vi "Main_State_Machine.vi"   [LabVIEW 2026]
uses:
  Typedefs/System_State.ctl
  Typedefs/BeltCtrl.ctl
  Globals.vi
types:
  T1 = enum16{"open", "replace", "create", "open or create", "replace or create", "replace or create with confirmation"}
  T2 = typedef "System_State.ctl" = u16
  T3 = typedef "BeltCtrl.ctl" = enum16{"Off", "Forward", "Back", "Coast", "Brake", ""}
  T4 = typedef "ServoCommand.ctl" = enum16{"colour 1", "Colour2", "Colour3", "Reject"}
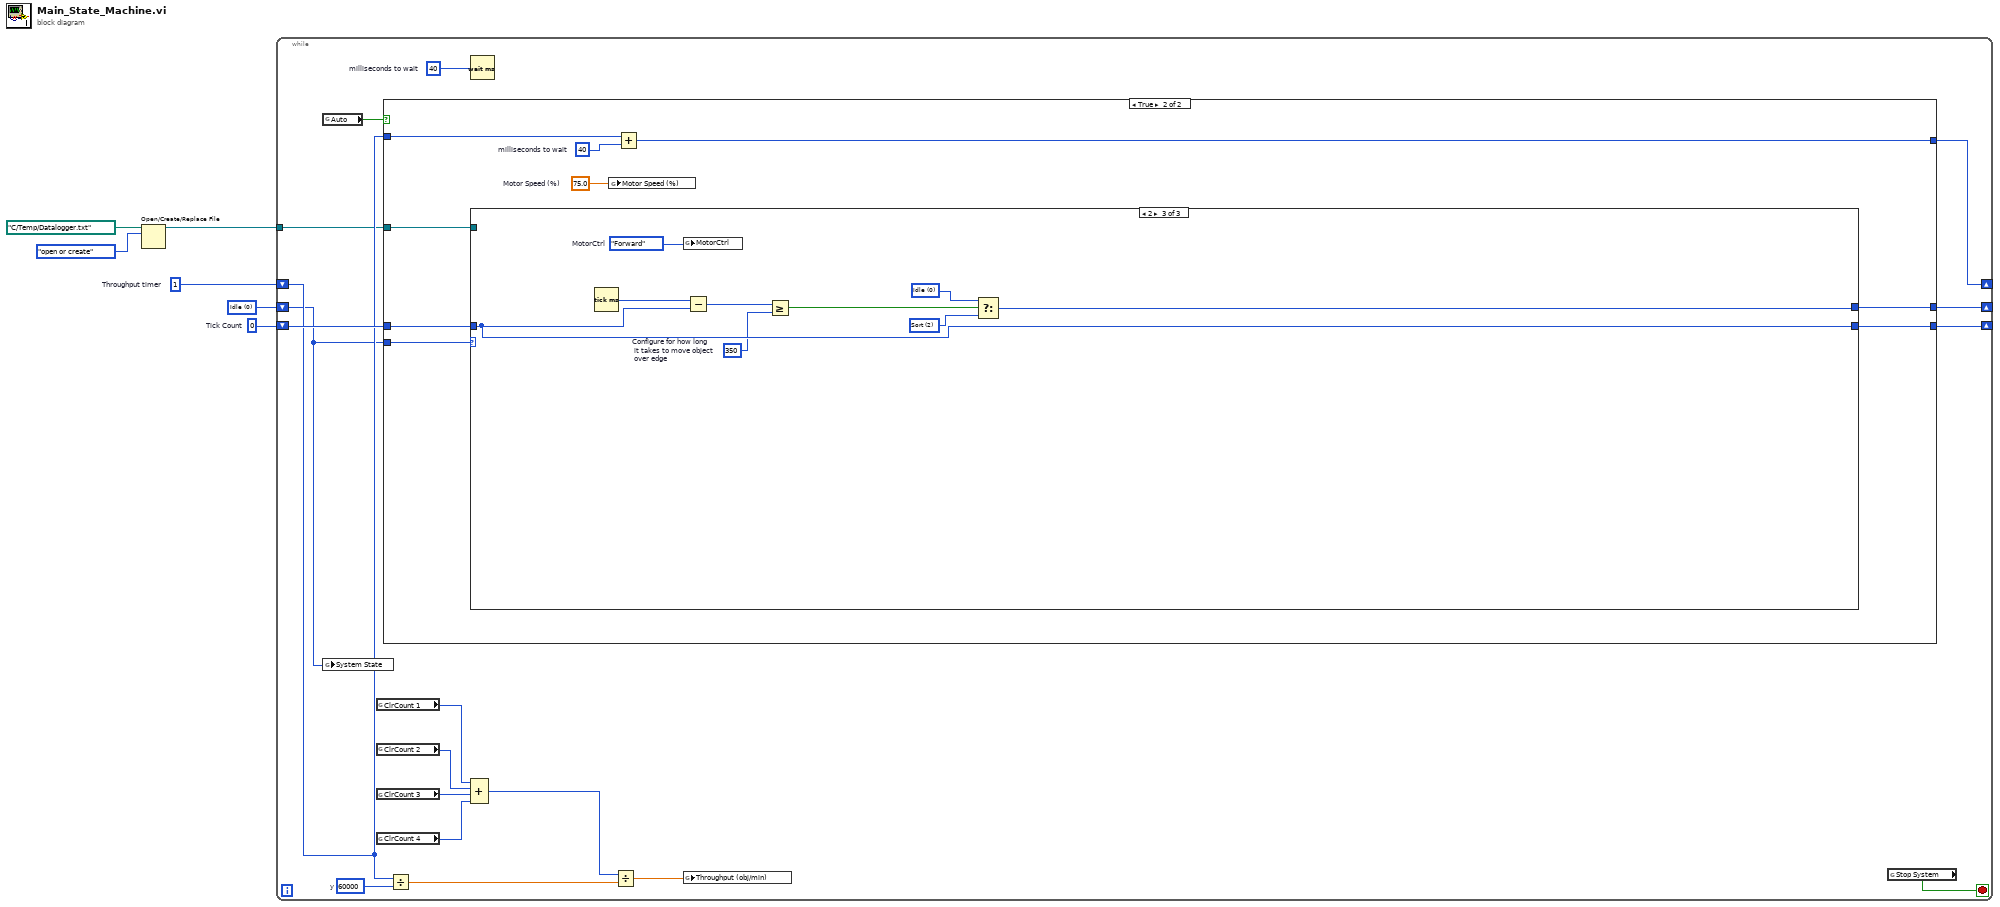
[diagram p0: block diagram]
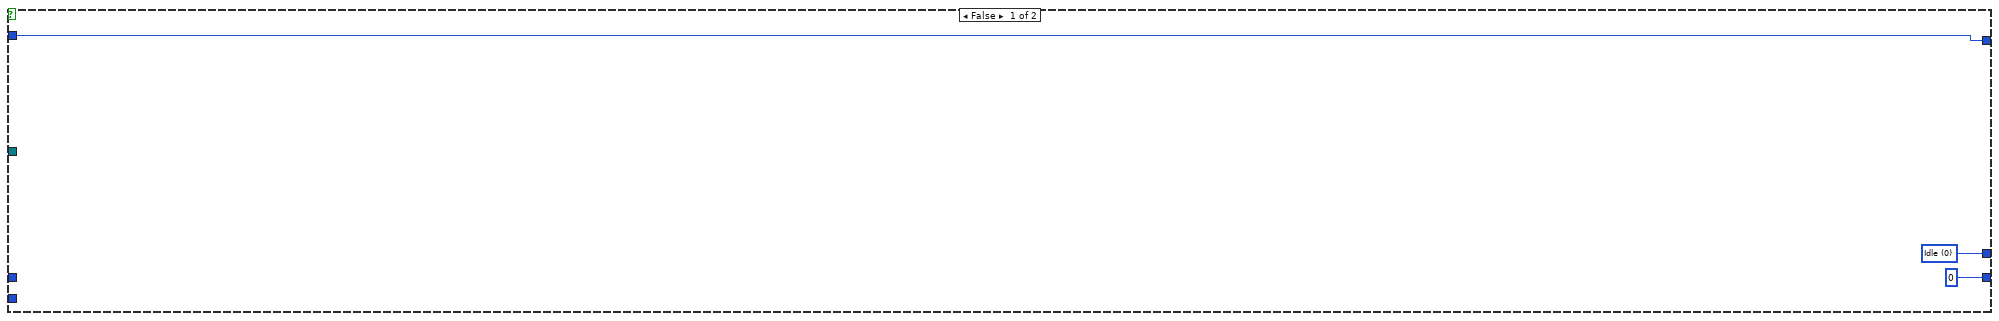
[diagram p2: hidden frame]
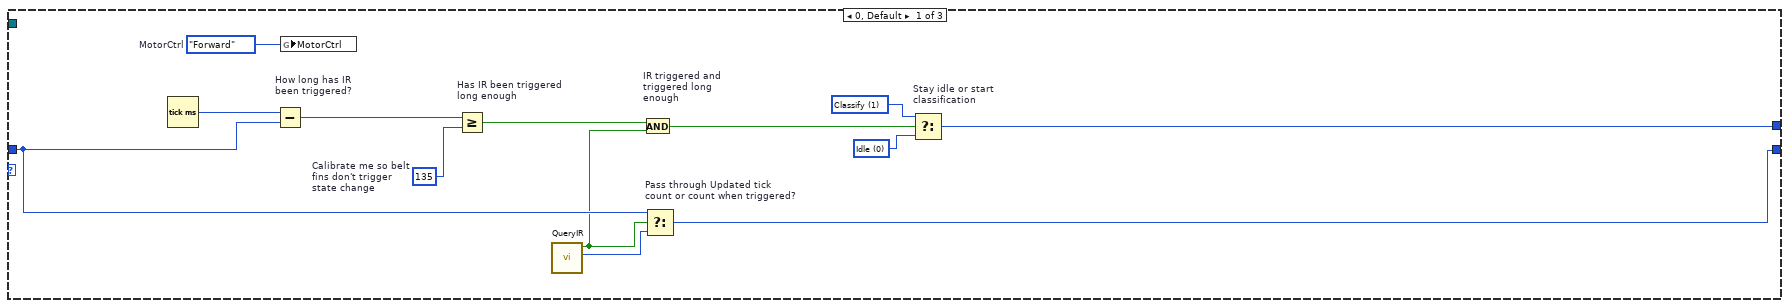
[diagram p3: hidden frame]
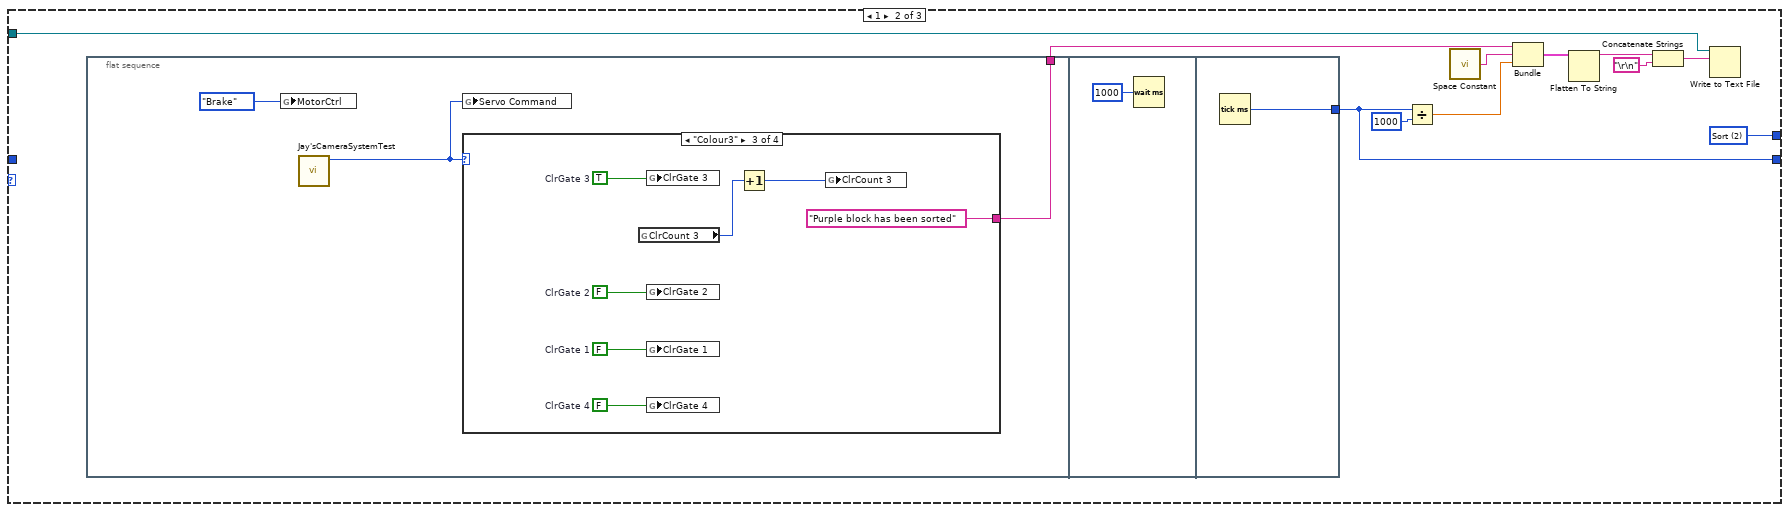
[diagram p4: hidden frame]
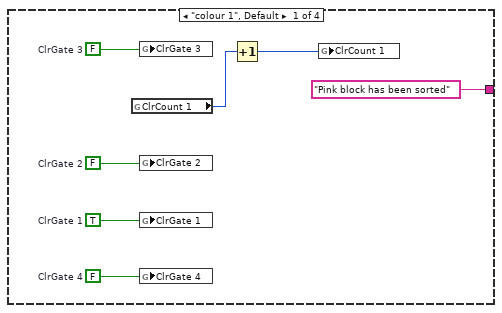
[diagram p5: hidden frame]
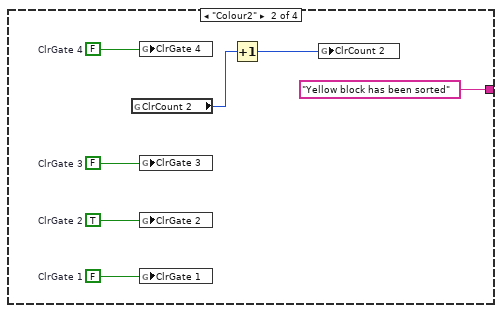
[diagram p6: hidden frame]
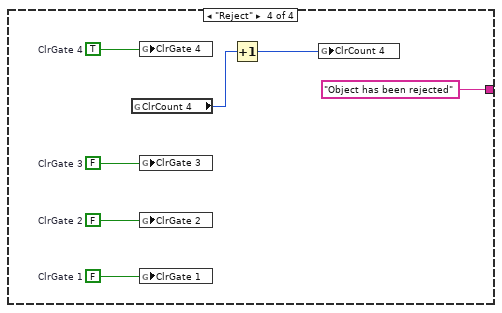
[diagram p7: hidden frame]
diagram:
  w2 = T2 0 items=["Idle", "Classify", "Sort"] ("System State")
  w5 = u32 1  # Throughput timer
  w6 = u32 0  # Tick Count
  n1 = Open/Create/Replace File(file path (use dialog)=path "C:/Temp/Datalogger.txt", operation (0:open)=T1."open or create") -> (refnum out=w4:refnum<file>)  [unwired: 4 in, 2 out]
  n2 = while {
    shift-right: [w24] -> _
    shift-left: w2 -> [w7]
    shift-right: [w21] -> _
    shift-left: w6 -> [w20]
    shift-right: [w10] -> _
    shift-left: w5 -> [w9]
    tunnel: w4 -> [w8]
    stop <- w23 stop-if-true
    w13 = u32 60000  # y
    w22 = u32 40  # milliseconds to wait
    n3 = global read "Globals.vi" "Auto"() -> (w19:bool)
    n4 = global write "Globals.vi" "System State"(w7) -> ()
    n5 = global read "Globals.vi" "ClrCount 1"() -> (w18:i32)
    n6 = global read "Globals.vi" "ClrCount 2"() -> (w17:i32)
    n7 = global read "Globals.vi" "ClrCount 3"() -> (w16:i32)
    n8 = global read "Globals.vi" "ClrCount 4"() -> (w15:i32)
    n9 = case shown="True" w19 {
      tunnel: [w25 w36] -> w24
      tunnel: [u32 0 ("millisecond timer value") w35] -> w21
      tunnel: w20 -> [_ w34]
      tunnel: w9 -> [w26 w33]
      tunnel: [w26 w31] -> w10
      tunnel: w8 -> [_ w29]
      tunnel: w7 -> [_ w28]
      frame False {
        w25 = T2 0 items=["Idle", "Classify", "Sort"] ("System State")
      }
      frame True {
        w30 = 75.0  # Motor Speed (%)
        w32 = u32 40  # milliseconds to wait
        n10 = case shown="2" w28 {
          tunnel: [w49 w50 w97] -> w36
          tunnel: [w45 w53 w101] -> w35
          tunnel: w34 -> [w43 _ w101]
          tunnel: w29 -> [_ w60 _]
          frame 0, Default {
            w37 = T2 0 items=["Idle", "Classify", "Sort"] ("System State")
            w38 = T2 1 items=["Idle", "Classify", "Sort"] ("System State")
            w39 = BeltCtrl."Forward"  # MotorCtrl
            w46 = u32 135  # Calibrate me so belt fins don't trigger  state change
            n11 = Tick Count (ms)() -> (millisecond timer value=w48:u32)
            n12 = Subtract "How long has IR\nbeen triggered?"(x=w48, y=w43) -> (x-y=w47:u32)
            n13 = global write "Globals.vi" "MotorCtrl"(w39) -> ()
            n14 = Greater Or Equal? "Has IR been triggered \nlong enough"(x=w47, y=w46) -> (x >= y?=w42:bool)
            n15 = call "QueryIR.vi"() -> ("Tick Count"=w44:u32, "Is there an object?"=w41:bool)  [unwired: 8 in]
            n16 = And "IR triggered and \ntriggered long \nenough"(x=w42, y=w41) -> (x .and. y?=w40:bool)
            n17 = Select "Pass through Updated tick\ncount or count when triggered?"(t=w43, s=w41, f=w44) -> (s? t:f=w45:u32)
            n18 = Select "Stay idle or start\nclassification"(t=w38, s=w40, f=w37) -> (s? t:f=w49:T2)
          }
          frame 1 {
            w50 = T2 2 items=["Idle", "Classify", "Sort"] ("System State")
            n19 = flat-sequence {
              tunnel: [w61] -> w58
              tunnel: [w93] -> w53
              frame #0 {
                n20 = global write "Globals.vi" "MotorCtrl"(BeltCtrl."Brake" ("MotorCtrl")) -> ()
                n21 = call "Jay'sCameraSystemTest.vi"() -> ("Servo Command"=w63:T4)  [unwired: 11 in]
                n22 = global write "Globals.vi" "Servo Command"(w63) -> ()
                n23 = case shown="\"Colour3\"" w63 {
                  tunnel: ["Pink block has been sorted" "Yellow block has been sorted" "Purple block has been sorted" "Object has been rejected"] -> w61
                  frame "colour 1", Default {
                    w68 = TRUE  # ClrGate 1
                    w67 = FALSE  # ClrGate 2
                    w66 = FALSE  # ClrGate 3
                    w65 = FALSE  # ClrGate 4
                    n24 = global read "Globals.vi" "ClrCount 1"() -> (w70:i32)
                    n25 = global write "Globals.vi" "ClrGate 3"(w66) -> ()
                    n26 = global write "Globals.vi" "ClrGate 2"(w67) -> ()
                    n27 = global write "Globals.vi" "ClrGate 1"(w68) -> ()
                    n28 = global write "Globals.vi" "ClrGate 4"(w65) -> ()
                    n29 = Increment(x=w70) -> (x+1=w69:i32)
                    n30 = global write "Globals.vi" "ClrCount 1"(w69) -> ()
                  }
                  frame "Colour2" {
                    w75 = FALSE  # ClrGate 1
                    w74 = TRUE  # ClrGate 2
                    w73 = FALSE  # ClrGate 3
                    w72 = FALSE  # ClrGate 4
                    n31 = global read "Globals.vi" "ClrCount 2"() -> (w77:i32)
                    n32 = global write "Globals.vi" "ClrGate 4"(w72) -> ()
                    n33 = global write "Globals.vi" "ClrGate 3"(w73) -> ()
                    n34 = global write "Globals.vi" "ClrGate 2"(w74) -> ()
                    n35 = global write "Globals.vi" "ClrGate 1"(w75) -> ()
                    n36 = Increment(x=w77) -> (x+1=w76:i32)
                    n37 = global write "Globals.vi" "ClrCount 2"(w76) -> ()
                  }
                  frame "Colour3" {
                    w82 = FALSE  # ClrGate 1
                    w81 = FALSE  # ClrGate 2
                    w80 = TRUE  # ClrGate 3
                    w79 = FALSE  # ClrGate 4
                    n38 = global read "Globals.vi" "ClrCount 3"() -> (w84:i32)
                    n39 = global write "Globals.vi" "ClrGate 3"(w80) -> ()
                    n40 = global write "Globals.vi" "ClrGate 2"(w81) -> ()
                    n41 = global write "Globals.vi" "ClrGate 1"(w82) -> ()
                    n42 = global write "Globals.vi" "ClrGate 4"(w79) -> ()
                    n43 = Increment(x=w84) -> (x+1=w83:i32)
                    n44 = global write "Globals.vi" "ClrCount 3"(w83) -> ()
                  }
                  frame "Reject" {
                    w89 = FALSE  # ClrGate 1
                    w88 = FALSE  # ClrGate 2
                    w87 = FALSE  # ClrGate 3
                    w86 = TRUE  # ClrGate 4
                    n45 = global read "Globals.vi" "ClrCount 4"() -> (w91:i32)
                    n46 = global write "Globals.vi" "ClrGate 4"(w86) -> ()
                    n47 = global write "Globals.vi" "ClrGate 3"(w87) -> ()
                    n48 = global write "Globals.vi" "ClrGate 2"(w88) -> ()
                    n49 = global write "Globals.vi" "ClrGate 1"(w89) -> ()
                    n50 = Increment(x=w91) -> (x+1=w90:i32)
                    n51 = global write "Globals.vi" "ClrCount 4"(w90) -> ()
                  }
                }
              }
              frame #1 {
                n52 = Wait (ms)(milliseconds to wait=u32 1000) -> ()  [unwired: 1 out]
              }
              frame #2 {
                n53 = Tick Count (ms)() -> (millisecond timer value=w93:u32)
              }
            }
            n54 = Divide(x=w53, y=1000) -> (x/y=w51:dbl)
            n55 = call <vilib>:"Space Constant.vi"() -> ("String"=w57:string)
            n56 = Bundle(w58, "String"=w57, w51) -> (w56:cluster{string, "String":string, dbl})  [unwired: 1 in]
            n57 = Flatten To String(anything=w56) -> (data string=w55:string)  [unwired: 3 in, 2 out]
            n58 = Concatenate Strings(w55, "\r\n") -> (w54:string)
            n59 = Write to Text File(file (use dialog)=w60, text=w54) -> ()  [unwired: 2 in, 3 out]
          }
          frame 2 {
            w94 = T2 2 items=["Idle", "Classify", "Sort"] ("System State")
            w95 = T2 0 items=["Idle", "Classify", "Sort"] ("System State")
            w96 = BeltCtrl."Forward"  # MotorCtrl
            w99 = u32 350  # Configure for how long  it takes to move object  over edge
            n60 = Tick Count (ms)() -> (millisecond timer value=w102:u32)
            n61 = global write "Globals.vi" "MotorCtrl"(w96) -> ()
            n62 = Subtract(x=w102, y=w101) -> (x-y=w100:u32)
            n63 = Greater Or Equal?(x=w100, y=w99) -> (x >= y?=w98:bool)
            n64 = Select(t=w95, s=w98, f=w94) -> (s? t:f=w97:T2)
          }
        }
        n65 = global write "Globals.vi" "Motor Speed (%)"(w30) -> ()
        n66 = Add(x=w33, y=w32) -> (x+y=w31:u32)
      }
    }
    n67 = Divide(x=w9, y=w13) -> (x/y=w12:dbl)
    n68 = Wait (ms)(milliseconds to wait=w22) -> ()  [unwired: 1 out]
    n69 = Compound Arithmetic op=ADD(w18, w17, w16, w15) -> (w14:i32)
    n70 = Divide(x=w14, y=w12) -> (x/y=w11:dbl)
    n71 = global write "Globals.vi" "Throughput (obj/min)"(w11) -> ()
    n72 = global read "Globals.vi" "Stop System"() -> (w23:bool)
  }
